vi "Set Warmup Data.vi"(8 "error in (no error)":errorcluster, 9 "Digital":u8[][](array[numeric]), 10 "Analog":dbl[][](array[numeric]), 11 "DAQ Timed SPIM in":refnum<class "DAQ Timed SPIM.lvclass">) -> (0 "error out":errorcluster, 3 "DAQ Timed SPIM out":refnum<class "DAQ Timed SPIM.lvclass">)   [LabVIEW 2020, in "DAQ Timed SPIM.lvlib" / "DAQ Timed SPIM.lvclass"]
uses:
  DAQ Timed SPIM.lvclass
  DAQ Timed SPIM.lvclass/DAQ Timed SPIM.ctl
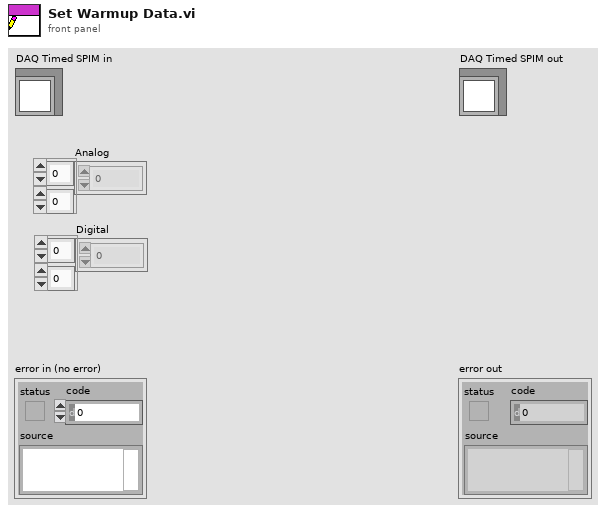
[diagram p1: front panel]
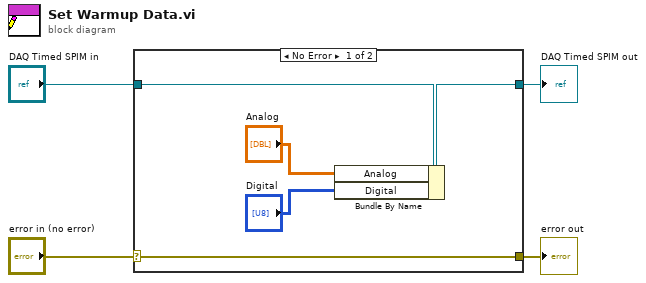
[diagram p0: block diagram]
diagram:
  n1 = case shown="No Error" "error in (no error)" {
    selector: "error in (no error)" -> [w9 w10]
    tunnel: [w9 w10] -> w3
    tunnel: [w7 w11] -> w1
    tunnel: "DAQ Timed SPIM in" -> [w8 w11]
    frame No Error {
      n2 = Bundle By Name(cluster=w8, "Analog"="Analog", "Digital"="Digital") -> (w7:refnum<class "DAQ Timed SPIM.lvclass">)
    }
    frame Error {
    }
  }
  "error out" <- w3
  "DAQ Timed SPIM out" <- w1
